vi "Caller.vi"(11 "error in":errorcluster) -> (15 "error out":errorcluster)   [LabVIEW 2026]
doc: "Issue 136 enum example: two enum typedef constants, State at Stop and Mode at Run."
uses:
  State.ctl
  Mode.ctl
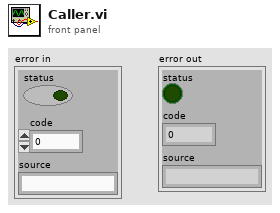
[diagram p1: front panel]
types:
  T1 = typedef "Mode.ctl" = enum16{"Off", "Run", "Stop"}
  T2 = typedef "State.ctl" = enum16{"Init", "Run", "Stop"}
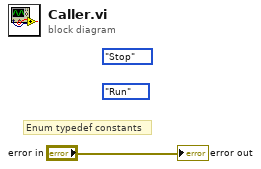
[diagram p0: block diagram]
diagram:
  (unwired) Mode."Run" ("Mode")
  (unwired) State."Stop" ("State")
  # "Enum typedef constants"
  "error out" <- "error in"
